vi "parseResult_getCharacters.vi"(0 "ocr in":refnum<class "ocr.lvclass">, 1 "numberofImgs":i32, 2 "totalTxt":i32, 4 "TextDecRecResult2L":T3[](array[typedef]), 5 "chars":u8[](array[numeric]), 7 "error in (no error)":errorcluster) -> (20 "ocr out":refnum<class "ocr.lvclass">, 22 "OCRResult":T1[](array[typedef]), 24 "!totalTxt mismatch":bool, 27 "error out":errorcluster)   [LabVIEW 2025, in "adsOCR.lvlib" / "ocr.lvclass"]
uses:
  ocr.lvclass
  ocr.lvclass/ocr.ctl
  ocrDetection.ctl
  ocrImageResult.ctl
  0fef4b09-d6c5-4d73-8228-e75743b5b14a.vi
  TextDecRecResult2L.ctl
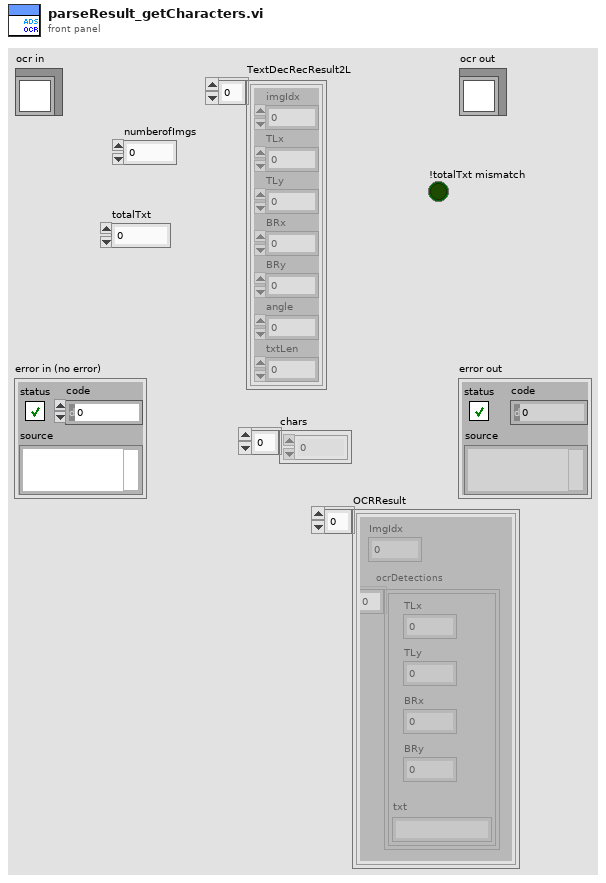
[diagram p1: front panel]
types:
  T1 = typedef "adsOCR.lvlib/ocr.lvclass/ocrImageResult.ctl" = cluster{"ImgIdx":i16, "ocrDetections":T2[]}
  T2 = typedef "adsOCR.lvlib/ocr.lvclass/ocrDetection.ctl" = cluster{"TLx":i32, "TLy":i32, "BRx":i32, "BRy":i32, "txt":string}
  T3 = typedef "adsOCR.lvlib/ocr.lvclass/TextDecRecResult2L.ctl" = cluster{"imgIdx":i32, "TLx":i32, "TLy":i32, "BRx":i32, "BRy":i32, "angle":sgl, "txtLen":i32}
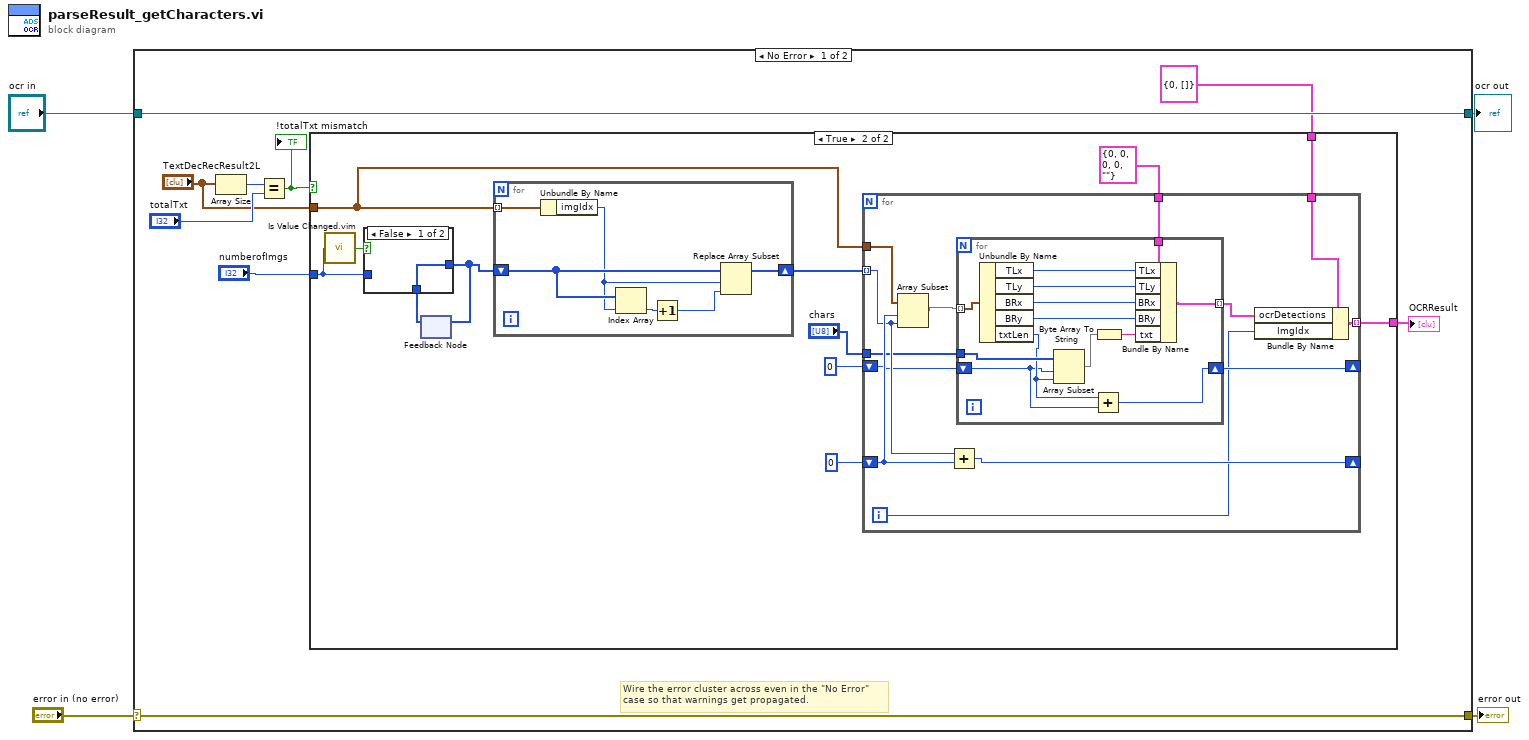
[diagram p0: block diagram]
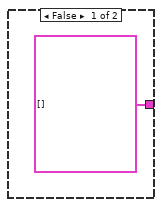
[diagram p2: hidden frame]
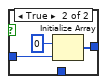
[diagram p3: hidden frame]
diagram:
  n1 = case shown="No Error" "error in (no error)" {
    selector: "error in (no error)" -> [w12 w64]
    tunnel: [w12 w64] -> w3
    tunnel: [w13 w63] -> w1
    tunnel: "ocr in" -> [w13 w63]
    frame No Error {
      # "Wire the error cluster across even in the \"No Error\"\ncase so that warnings get propagated."
      n2 = Array Size(array="TextDecRecResult2L") -> (size(s)=w10:i32)
      n3 = Equal?(x=w10, y="totalTxt") -> (x = y?=w9:bool)
      "!totalTxt mismatch" <- w9
      n4 = case shown="True" w9 {
        tunnel: "numberofImgs" -> [_ w24]
        tunnel: "TextDecRecResult2L" -> [_ w19]
        tunnel: T1 {"ImgIdx"=0, "ocrDetections"=[]} ("ocrImageResult") -> [_ w16]
        tunnel: [T1[] [] w15] -> w5
        frame False {
        }
        frame True {
          n5 = call "Is Value Changed.vim"("value"=w24) -> ("changed or first call?"=w25:bool)
          n6 = feedback #1() -> (w22:i32[])  [unwired: 1 in]
          n7 = case shown="False" w25 {
            tunnel: w24 -> [_ w30]
            tunnel: [w27 w28] -> w23
            tunnel: w22 -> [w27 _]
            frame False {
            }
            frame True {
              n8 = Initialize Array(0 ("element"), w30) -> (w28:i32[])
            }
          }
          n9 = feedback-in #1(w23) -> ()
          n10 = for {
            tunnel: w19 -> [w62] mode=indexing
            shift-right: [w57] -> w26
            shift-left: w23 -> [w60]
            n11 = Unbundle By Name(w62) -> ("imgIdx"=w59:i32)
            n12 = Index Array(array=w60, index=w59) -> (element=w61:i32)
            n13 = Increment(x=w61) -> (x+1=w58:i32)
            n14 = Replace Array Subset(array=w60, new element=w58, index=w59) -> (w57:i32[])
          }
          n15 = for {
            tunnel: w26 -> [w40] mode=indexing
            shift-right: [w37] -> _
            shift-left: 0 -> [w38]
            shift-right: [w39] -> _
            shift-left: 0 -> [w41]
            tunnel: w19 -> [w43]
            tunnel: "chars" -> [w36]
            tunnel: T2 {"TLx"=0, "TLy"=0, "BRx"=0, "BRy"=0, "txt"=""} ("ocrDetection") -> [w35]
            tunnel: w16 -> [w34]
            tunnel: [w31] -> w15 mode=indexing
            i -> [w32]
            n16 = Array Subset(array=w43, index=w41, length=w40) -> (w42:T3[])
            n17 = Add(x=w40, y=w41) -> (x+y=w39:i32)
            n18 = for {
              tunnel: w42 -> [w56] mode=indexing
              shift-right: [w51] -> w37
              shift-left: w38 -> [w52]
              tunnel: w36 -> [w55]
              tunnel: w35 -> [w50]
              tunnel: [w44] -> w33 mode=indexing
              n19 = Unbundle By Name(w56) -> ("TLx"=w49:i32, "TLy"=w48:i32, "BRx"=w47:i32, "BRy"=w46:i32, "txtLen"=w53:i32)
              n20 = Array Subset(array=w55, index=w52, length=w53) -> (w54:u8[])
              n21 = Add(x=w53, y=w52) -> (x+y=w51:i32)
              n22 = Byte Array To String(unsigned byte array=w54) -> (string=w45:string)
              n23 = Bundle By Name(cluster=w50, "TLx"=w49, "TLy"=w48, "BRx"=w47, "BRy"=w46, "txt"=w45) -> (w44:T2)
            }
            n24 = Bundle By Name(cluster=w34, "ocrDetections"=w33, "ImgIdx"=w32) -> (w31:T1)
          }
        }
      }
      "OCRResult" <- w5
    }
    frame Error {
    }
  }
  "error out" <- w3
  "ocr out" <- w1
